vi "Comm_Step.vi"(4 "Host":string, 5 "Port":u16, 6 "COM Port":refnum<visa-resource-name>, 7 "error in (no error)":errorcluster, 8 "Transport":T1(ring), 9 "Connected":bool, 10 "PLC Conn":refnum<visa-resource-name>, 11 "Queue":refnum<queue>) -> (0 "Stop":bool, 1 "Words":u16[](array[numeric]), 2 "Connected out":bool, 3 "PLC Conn out":refnum<visa-resource-name>)   [LabVIEW 2026]
doc: "Use this template to build a VI to use as a subVI."
panel:
  # "ÕfÃ÷£ºÍ¨ÓÞÈ¦µÄÒ»È¦¡£ÒÑßB¾£ºÍêÐÁÐÃüÁîÔÙ×x±OÒÙYÁÏ¡£Î´ßB¾£ºÖØé_\n£¬KÇå¿ÕÐÁÐ£¬±ÜÃâÅfµÄücÓÃüÁîÔÚÖØßBáá²ÅËÍ³ö¡£"
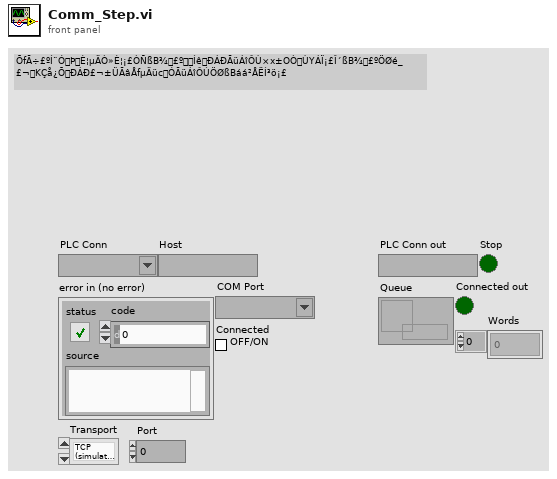
[diagram p1: front panel]
types:
  T1 = enum16{"TCP (simulator)", "RS-422 (COM)", "USB (COM)"}
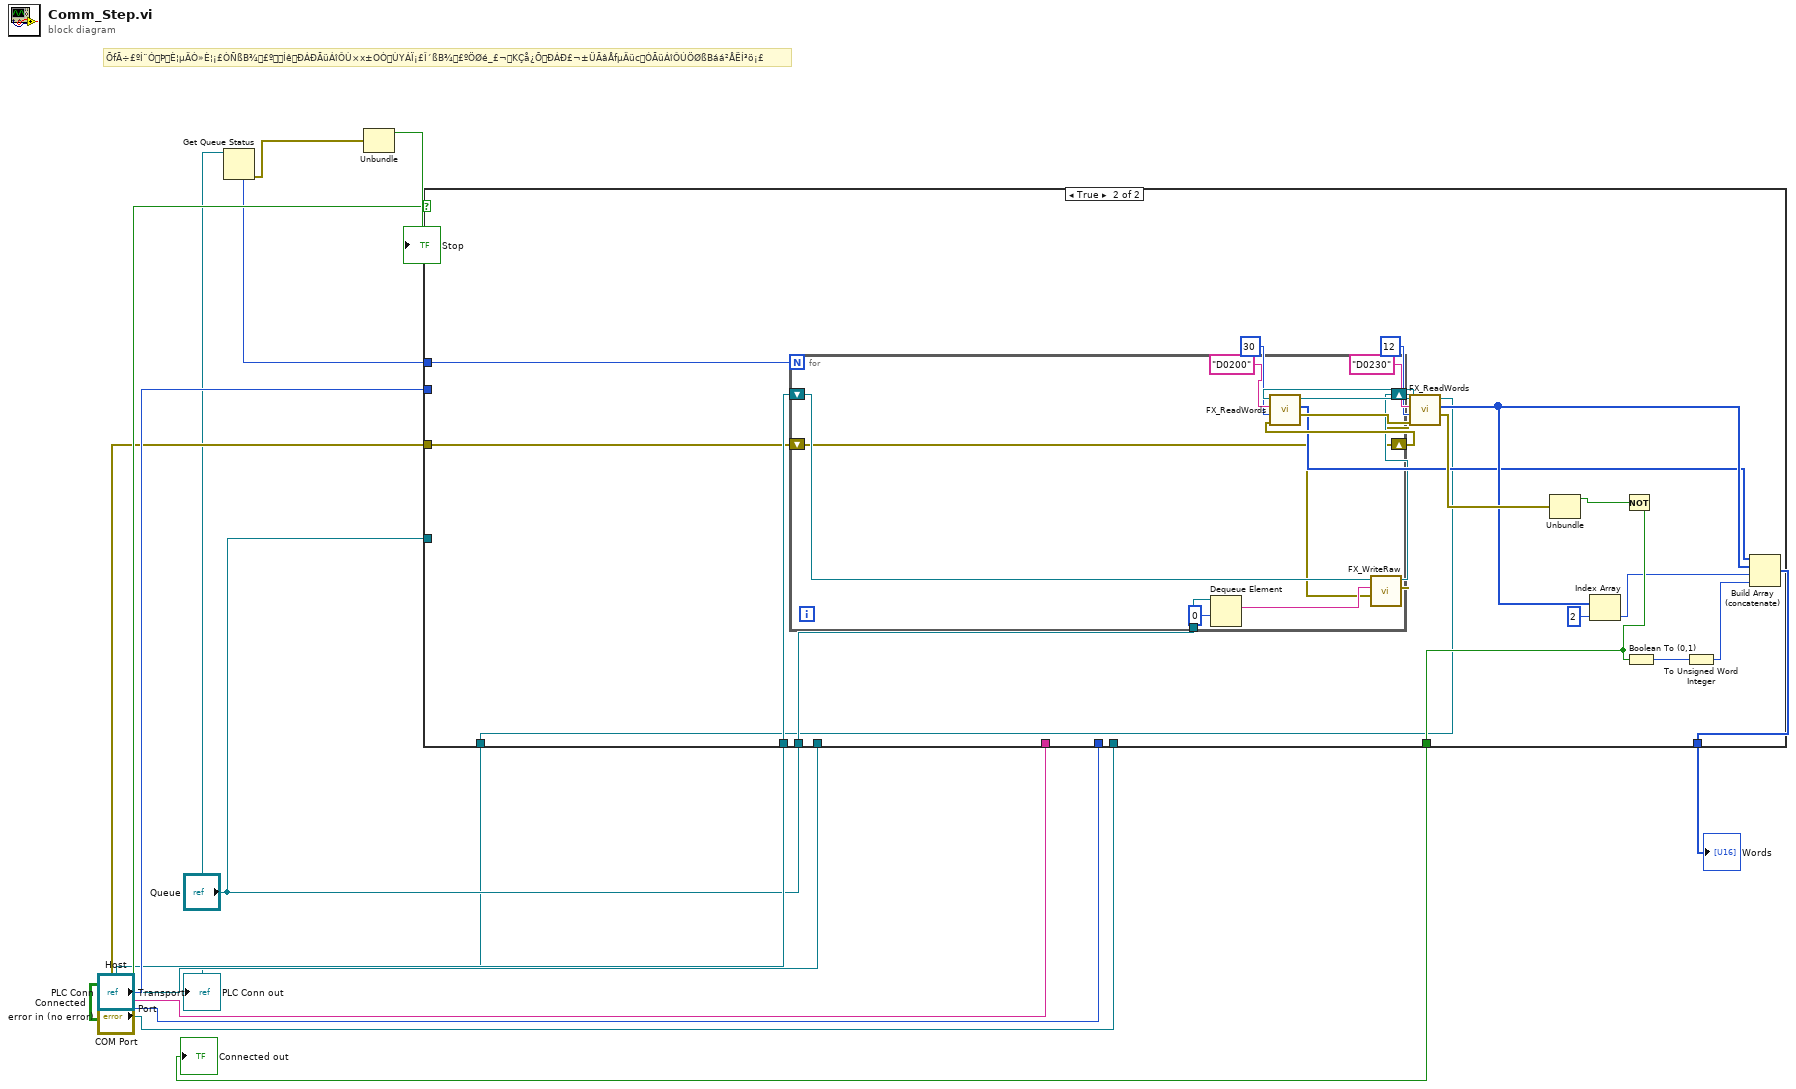
[diagram p0: block diagram]
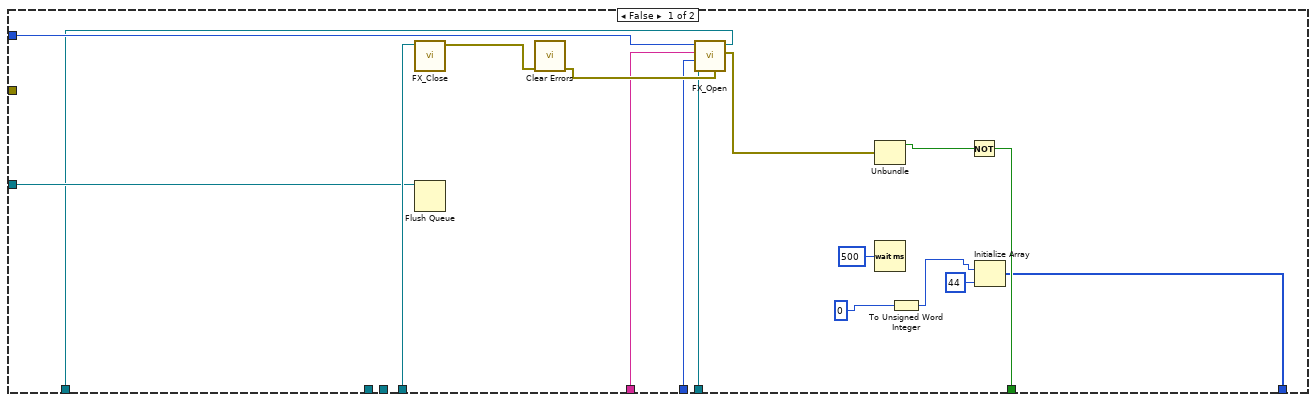
[diagram p2: hidden frame]
diagram:
  # "ÕfÃ÷£ºÍ¨ÓÞÈ¦µÄÒ»È¦¡£ÒÑßB¾£ºÍêÐÁÐÃüÁîÔÙ×x±OÒÙYÁÏ¡£Î´ßB¾£ºÖØé_£¬KÇå¿ÕÐÁÐ£¬±ÜÃâÅfµÄücÓÃüÁîÔÚÖØßBáá²ÅËÍ³ö¡£"
  n1 = Get Queue Status(queue="Queue") -> (error out=w14:errorcluster, # elements in queue=w7:i32)  [unwired: 2 in, 6 out]
  n2 = Unbundle(w14) -> ("status"=→"Stop":bool)  [unwired: 2 out]
  n3 = case shown="True" "Connected" {
    tunnel: "PLC Conn" -> [w31 _]
    tunnel: "Queue" -> [w29 _]
    tunnel: "Transport" -> [w27 _]
    tunnel: "Host" -> [w26 _]
    tunnel: "Port" -> [w25 _]
    tunnel: "COM Port" -> [w24 _]
    tunnel: w7 -> [_ w54]
    tunnel: "PLC Conn" -> [_ w53]
    tunnel: "error in (no error)" -> [_ w52]
    tunnel: "Queue" -> [_ w51]
    tunnel: [w17 w33] -> w3
    tunnel: [w16 w38] -> w2
    tunnel: [w15 w32] -> w1
    frame False {
      n4 = call "FX_Close.vi"("PLC Conn"=w31) -> ("error out"=w30:errorcluster)  [unwired: 10 in]
      n5 = Flush Queue(queue=w29) -> ()  [unwired: 1 in, 3 out]
      n6 = call <vilib>:"Clear Errors.vi"("error in (no error)"=w30) -> ("error out"=w28:errorcluster)  [unwired: 5 in, 1 out]
      n7 = call "FX_Open.vi"("error in (no error)"=w28, "COM Port"=w24, "Port"=w25, "Host"=w26, "Transport"=w27) -> ("error out"=w23:errorcluster, "PLC Conn"=w17:refnum<visa-resource-name>)  [unwired: 5 in]
      n8 = Unbundle(w23) -> ("status"=w22:bool)  [unwired: 2 out]
      n9 = Wait (ms)(milliseconds to wait=u32 500) -> ()  [unwired: 1 out]
      n10 = To Unsigned Word Integer(number=0) -> (unsigned 16bit integer=w18:u16)
      n11 = Not(x=w22) -> (.not. x?=w16:bool)
      n12 = Initialize Array(w18, 44 ("dimension size")) -> (w15:u16[])
    }
    frame True {
      n13 = for {
        N: w54 -> [_]
        shift-right: [w56] -> w50
        shift-left: w53 -> [w58]
        shift-right: [w55] -> w49
        shift-left: w52 -> [w57]
        tunnel: w51 -> [w61]
        n14 = Dequeue Element(queue=w61, timeout in ms (-1)=0) -> (element=w59:string)  [unwired: 1 in, 3 out]
        n15 = call "FX_WriteRaw.vi"("error in (no error)"=w57, "Cmd"=w59, "PLC Conn"=w58) -> ("error out"=w55:errorcluster, "PLC Conn out"=w56:refnum<visa-resource-name>)  [unwired: 7 in]
      }
      n16 = call "FX_ReadWords.vi"("error in (no error)"=w49, "Count"=u16 30, "Device"="D0200", "PLC Conn"=w50) -> ("error out"=w45:errorcluster, "Words"=w36:u16[], "PLC Conn out"=w46:refnum<visa-resource-name>)  [unwired: 5 in]
      n17 = call "FX_ReadWords.vi"("error in (no error)"=w45, "Count"=u16 12, "Device"="D0230", "PLC Conn"=w46) -> ("error out"=w42:errorcluster, "Words"=w40:u16[], "PLC Conn out"=w33:refnum<visa-resource-name>)  [unwired: 5 in]
      n18 = Unbundle(w42) -> ("status"=w41:bool)  [unwired: 2 out]
      n19 = Index Array(array=w40, index=2) -> (element=w35:u16)
      n20 = Not(x=w41) -> (.not. x?=w38:bool)
      n21 = Boolean To (0,1)(Boolean=w38) -> (0, 1=w37:i16)
      n22 = To Unsigned Word Integer(number=w37) -> (unsigned 16bit integer=w34:u16)
      n23 = Build Array (concatenate)(w36, w40, w35, w34) -> (w32:u16[])
    }
  }
  "PLC Conn out" <- w3
  "Connected out" <- w2
  "Words" <- w1
